vi "Relay_num.vi"(0 "Relay_no.":dbl format="%#_13g") -> (2 "x = y?":bool, 3 "Relay":string[](array[string]), 4 "Relay_no.out":dbl format="%#_13g")   [LabVIEW 2025]
uses:
  Lamps_global.vi
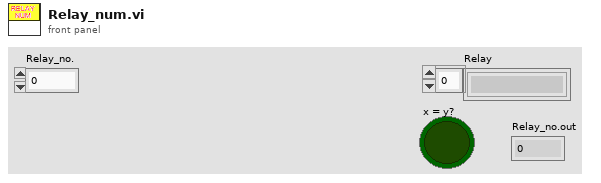
[diagram p1: front panel]
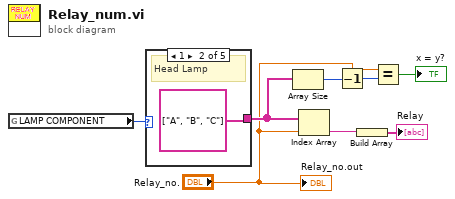
[diagram p0: block diagram]
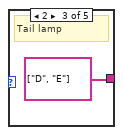
[diagram p3: hidden frame]
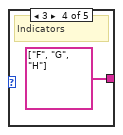
[diagram p4: hidden frame]
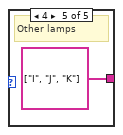
[diagram p5: hidden frame]
diagram:
  n1 = global read "Lamps_global.vi" "LAMP COMPONENT"() -> (w8:u16)
  n2 = case shown="1" w8 {
    tunnel: [_ string[] ["A", "B", "C"] string[] ["D", "E"] string[] ["F", "G", "H"] string[] ["I", "J", "K"]] -> w6
    frame 0, Default {
    }
    frame 1 {
      # "Head Lamp"
    }
    frame 2 {
      # "Tail lamp"
    }
    frame 3 {
      # "Indicators"
    }
    frame 4 {
      # "Other lamps"
    }
  }
  n3 = Array Size(array=w6) -> (size(s)=w3:i32)
  n4 = Index Array(array=w6, index="Relay_no.") -> (element=w7:string)
  n5 = Decrement(x=w3) -> (x-1=w2:i32)
  n6 = Build Array(w7) -> (→"Relay":string[])
  n7 = Equal?(x="Relay_no.", y=w2) -> (x = y?=→"x = y?":bool)
  "Relay_no.out" <- "Relay_no."
